vi "fake prompt ask user.vi"() -> (0 "error out":errorcluster, 3 "resulting string":string)   [LabVIEW 2020, in "MCP Server tests.lvlib"]
doc: "Fake prompt to test elicitation in prompts/get (MCP 2026-07-28). It asks \"What context should the prompt use?\" with Ask User.vi (key context, a form with the string property context) and returns the text \"Use this context: <context>\". While the question is pending it returns at once."
uses:
  MCP Server tests.lvlib
  <vilib>/JDP Science/JSONtext/Next JSON Value.vi
  <vilib>/JDP Science/JSONtext/String Subset.vi
  <vilib>/JDP Science/JSONtext/support/Strip Quotes and Unescape.vi
  <vilib>/JDP Science/JSONtext/Parsing/Advance past next JSON Value (inlined COPY).vi
  <vilib>/JDP Science/JSONtext/support/Unescape JSON string.vi
  <vilib>/JDP Science/JSONtext/Parsing/Advance past whitespace.vi
  <vilib>/JDP Science/JSONtext/Parsing/Advance past String.vi
  <vilib>/JDP Science/JSONtext/Parsing/Advance past Number.vi
  <vilib>/JDP Science/JSONtext/Parsing/Advance past Line Ending.vi
  <vilib>/JDP Science/JSONtext/Parsing/Parse Full Path or Item Name.vi
  <vilib>/JDP Science/JSONtext/Parsing/Advance past Array.vi
  <vilib>/JDP Science/JSONtext/Parsing/Advance past Object.vi
  <vilib>/JDP Science/JSONtext/support/Error Cluster From Code.vi
  <vilib>/JDP Science/JSONtext/Offset/Find Item Locations by Path.vi
  <vilib>/JDP Science/JSONtext/Parsing/Advance past next JSON Value.vi
  src/MCP Server/MCP Server.lvlib
  <vilib>/JDP Science/JSONtext/JSONtext.lvlib
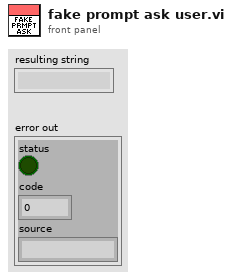
[diagram p1: front panel]
types:
  T1 = enum16{"accept", "decline", "cancel", "pending", "not supported"}
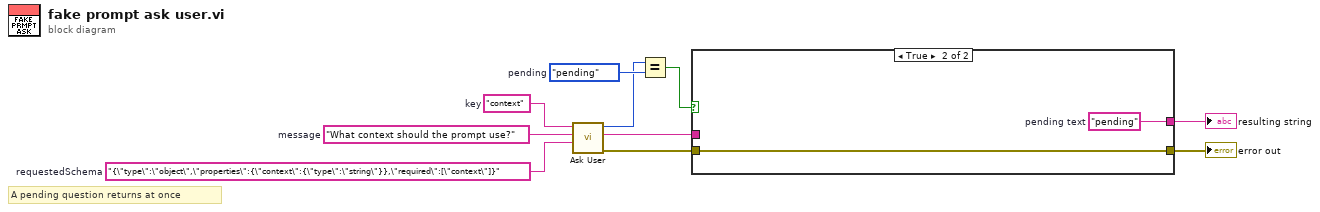
[diagram p0: block diagram]
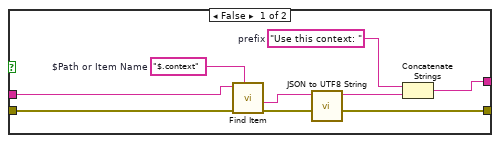
[diagram p2: hidden frame]
diagram:
  w7 = T1."pending"  # pending
  w3 = "{\"type\":\"object\",\"properties\":{\"context\":{\"type\":\"string\"}},\"required\":[\"context\"]}"  # requestedSchema
  w2 = "What context should the prompt use?"  # message
  w1 = "context"  # key
  # "A pending question returns at once"
  n1 = call "Ask User.vi"("requestedSchema"=w3, "message"=w2, "key"=w1) -> ("error out"=w6:errorcluster, "content"=w5:string, "action"=w4:T1)  [unwired: 6 in]
  n2 = Equal?(x=w4, y=w7) -> (x = y?=w8:bool)
  n3 = case shown="True" w8 {
    tunnel: [w19 w21] -> w9
    tunnel: w5 -> [w11 _]
    tunnel: w6 -> [w12 w20]
    tunnel: [w17 w20] -> w10
    frame False {
      w18 = "Use this context: "  # prefix
      w13 = "$.context"  # $Path or Item Name
      n4 = call <vilib>:"Find Item.vi"("$Path or Item Name"=w13, "error in (no error)"=w12, "JSON"=w11) -> ("error out"=w14:errorcluster, "<JSON>"=w15:string)  [unwired: 5 in, 2 out]
      n5 = call <vilib>:"JSON to UTF8 String.vi"("error in (no error)"=w14, "JSON"=w15) -> ("error out"=w17:errorcluster, "<UTF8>String"=w16:string)  [unwired: 8 in]
      n6 = Concatenate Strings(w18, w16) -> (w19:string)
    }
    frame True {
      w21 = "pending"  # pending text
    }
  }
  "resulting string" <- w9
  "error out" <- w10
